vi "Read move FP and BD.vi"(8 "error in":errorcluster, 11 "cosmetic changes in":refnum<class "cosmetic changes.lvclass">) -> (0 "error out":errorcluster, 2 "move FP and BD":bool, 3 "cosmetic changes out":refnum<class "cosmetic changes.lvclass">)   [LabVIEW 2013, in "cosmetic changes.lvclass"]
uses:
  cosmetic changes.lvclass
  cosmetic changes.lvclass/cosmetic changes.ctl
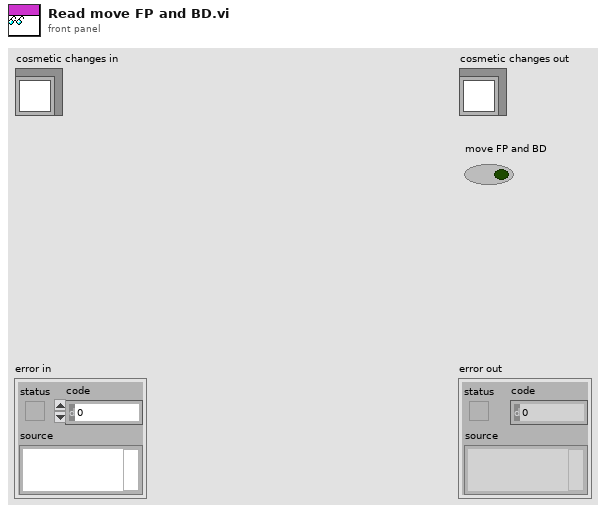
[diagram p1: front panel]
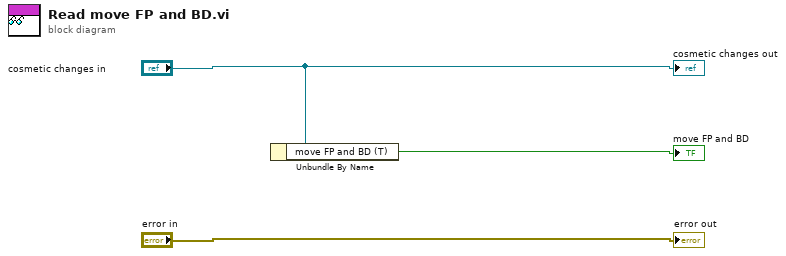
[diagram p0: block diagram]
diagram:
  n1 = Unbundle By Name("cosmetic changes in") -> ("move FP and BD (T)"=→"move FP and BD":bool)
  "error out" <- "error in"
  "cosmetic changes out" <- "cosmetic changes in"
